vi "SLSC Write Properties.vi"(0 "session in":refnum<k21>, 1 "Stop Updating?":bool, 3 "Detect?":bool[](array[boolean]), 5 "SLSC Module Name":refnum<k21>, 9 "Values":dbl[](array[numeric]), 11 "error in":errorcluster, 12 "SLSC Dynamic Outputs":T1[](array[typedef]), 13 "Change Commands":T1[](array[typedef]), 14 "Command Values":dbl[](array[numeric])) -> (4 "session out":refnum<k21>, 6 "SLSC Module Name":refnum<k21>, 8 "LoopRate(ms)":u32=50, 15 "error out":errorcluster)   [LabVIEW 2020, in "SLSC CD Engine.lvlib"]
uses:
  SLSC CD Engine.lvlib
  SLSC Dynamic Channel.ctl
  SLSC Datatype.ctl
  <vilib>/SLSC/Execute Command.vi
  <vilib>/SLSC/Execute Device Command.vi
  <vilib>/SLSC/Execute Phys Chan Command.vi
  <vilib>/SLSC/Commit Properties for Devices.vi
  <vilib>/SLSC/Set Generic Property (U64).vi
  <vilib>/SLSC/Set Generic Property (I64).vi
  <vilib>/SLSC/Set Generic Property (Bool).vi
  <vilib>/SLSC/Set Generic Property (String).vi
  <vilib>/SLSC/Set Generic Property (U32).vi
  <vilib>/SLSC/Set Generic Property (I32).vi
  <vilib>/SLSC/Set Generic Property (DBL).vi
  <vilib>/SLSC/SLSC.lvlib
  SLSC CD Shared/SLSC CD Shared.lvlib
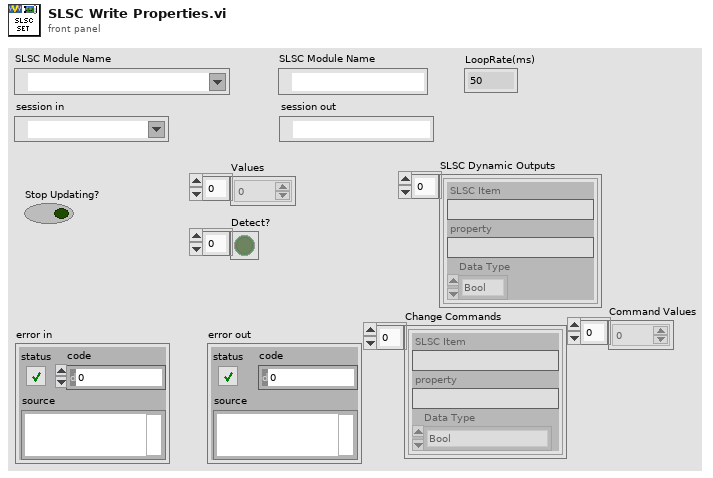
[diagram p1: front panel]
types:
  T1 = typedef "SLSC CD Shared.lvlib/SLSC Dynamic Channel.ctl" = cluster{"SLSC Item":string, "property":string, "Data Type":T2}
  T2 = typedef "SLSC CD Shared.lvlib/SLSC Datatype.ctl" = enum16{"Bool", "Double", "I32", "I64", "String", "U32", "U64"}
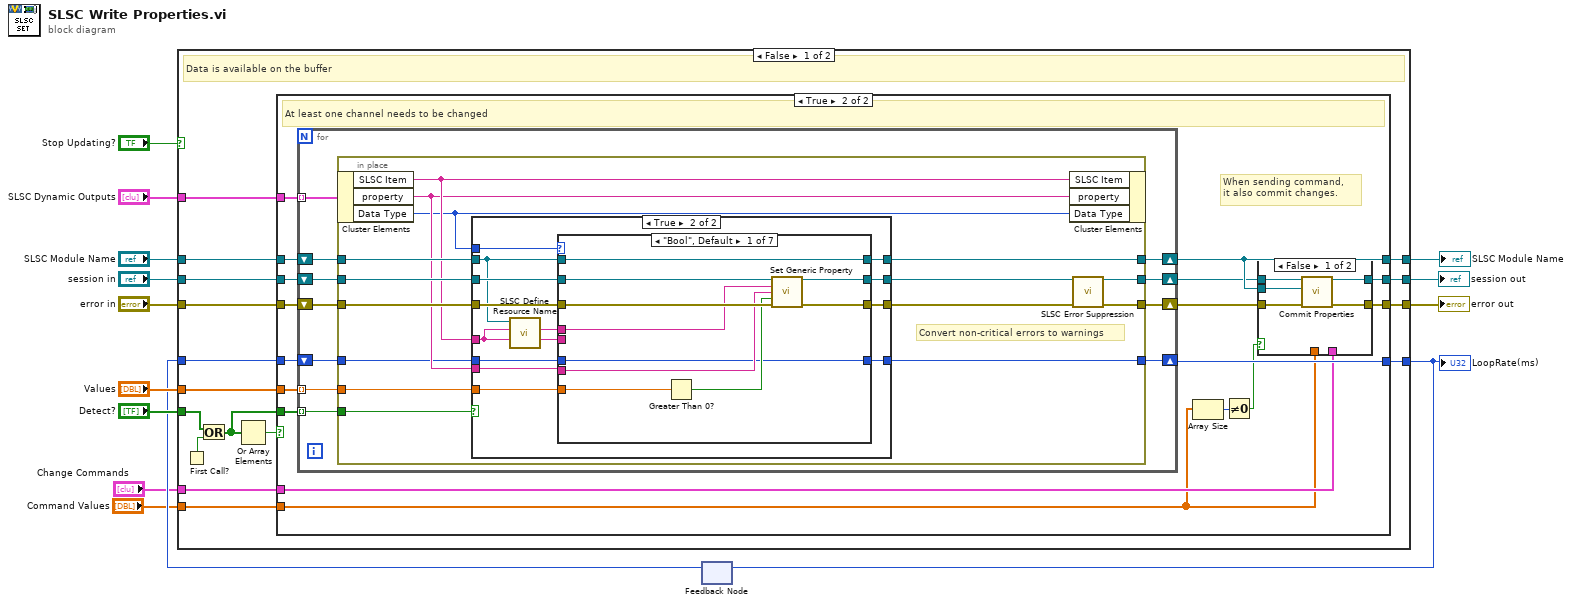
[diagram p0: block diagram]
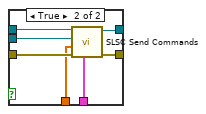
[diagram p3: hidden frame]
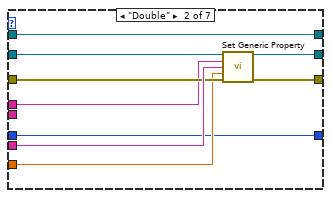
[diagram p5: hidden frame]
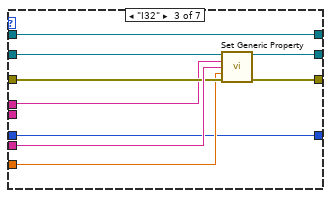
[diagram p6: hidden frame]
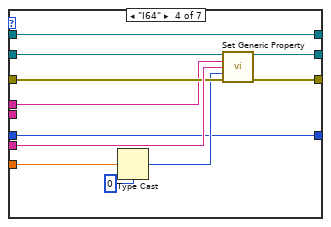
[diagram p7: hidden frame]
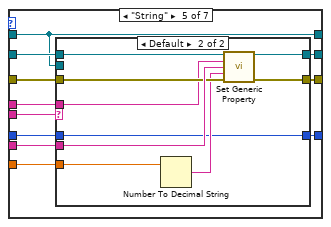
[diagram p8: hidden frame]
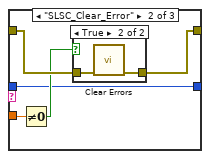
[diagram p10: hidden frame]
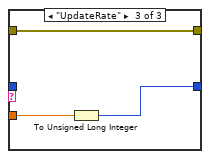
[diagram p12: hidden frame]
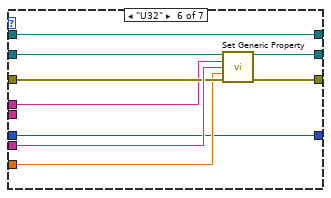
[diagram p13: hidden frame]
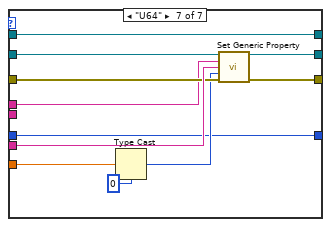
[diagram p14: hidden frame]
diagram:
  n1 = feedback #1() -> (w3:u32)  [unwired: 1 in]
  n2 = case shown="False" "Stop Updating?" {
    tunnel: "error in" -> [w30 w206]
    tunnel: "SLSC Dynamic Outputs" -> [w29 _]
    tunnel: "Values" -> [w28 _]
    tunnel: "session in" -> [w27 w207]
    tunnel: "SLSC Module Name" -> [w26 w208]
    tunnel: [w20 w208] -> w10
    tunnel: [w25 w206] -> w9
    tunnel: [w24 w207] -> w8
    tunnel: "Detect?" -> [w23 _]
    tunnel: [w21 w205] -> w4
    tunnel: w3 -> [w22 w205]
    tunnel: "Change Commands" -> [w18 _]
    tunnel: "Command Values" -> [w17 _]
    frame False {
      # "Data is available on the buffer"
      n3 = First Call?() -> (First Call?: T/F=w15:bool)
      n4 = Or(x=w23, y=w15) -> (x .or. y?=w16:bool[])
      n5 = Or Array Elements(Boolean array=w16) -> (logical OR=w19:bool)
      n6 = case shown="True" w19 {
        tunnel: w30 -> [w32 w51]
        tunnel: w29 -> [_ w50]
        tunnel: w28 -> [_ w49]
        tunnel: w27 -> [w33 w48]
        tunnel: w26 -> [w34 w47]
        tunnel: [w32 w42] -> w25
        tunnel: [w33 w43] -> w24
        tunnel: w16 -> [_ w46]
        tunnel: w22 -> [w31 w45]
        tunnel: [w31 w44] -> w21
        tunnel: [w34 w41] -> w20
        tunnel: w18 -> [_ w40]
        tunnel: w17 -> [_ w35]
        frame False {
          # "Do change detected, bypass write action"
        }
        frame True {
          # "When sending command,\nit also commit changes."
          # "At least one channel needs to be changed"
          n7 = for {
            tunnel: w49 -> [w74] mode=indexing
            tunnel: w50 -> [w67] mode=indexing
            shift-right: [w72] -> w36
            shift-left: w48 -> [w73]
            shift-right: [w71] -> w41
            shift-left: w47 -> [w68]
            tunnel: w46 -> [w66] mode=indexing
            shift-right: [w64] -> w44
            shift-left: w45 -> [w65]
            shift-right: [w69] -> w37
            shift-left: w51 -> [w70]
            n8 = in-place {
              in-place-border: w74 -> [w80]
              in-place-border: w73 -> [w88]
              in-place-border: [w87] -> w72
              in-place-border: [w86] -> w71
              in-place-border: w70 -> [w85]
              in-place-border: [w75] -> w69
              in-place-border: w68 -> [w84]
              in-place-border: w66 -> [w79]
              in-place-border: [w77] -> w64
              in-place-border: w65 -> [w76]
              # "Convert non-critical errors to warnings"
              n9 = in-place-cluster #2(w67) -> ("SLSC Item"=w83:string, "property"=w82:string, "Data Type"=w81:T2)
              n10 = case shown="True" w79 {
                tunnel: w88 -> [w91 w105]
                tunnel: [w91 w104] -> w87
                tunnel: [w92 w103] -> w86
                tunnel: w85 -> [w90 w102]
                tunnel: [w90 w101] -> w78
                tunnel: w84 -> [w92 w100]
                tunnel: w83 -> [_ w98]
                tunnel: w82 -> [_ w97]
                tunnel: w81 -> [_ w96]
                tunnel: w80 -> [_ w95]
                tunnel: [w89 w94] -> w77
                tunnel: w76 -> [w89 w93]
                frame False {
                }
                frame True {
                  n11 = call "SLSC Define Resource Name.vi"("SLSC Item"=w98, "SLSC Module Name"=w100) -> ("Resource"=w99:string)  [unwired: 9 in]
                  n12 = case shown="\"Bool\", Default" w96 {
                    tunnel: w95 -> [w110 w118 w127 w138 w150 w187 w197]
                    tunnel: w105 -> [w115 w124 w133 w144 w155 w193 w204]
                    tunnel: [w114 w123 w132 w143 w154 w192 w203] -> w104
                    tunnel: w97 -> [w107 w122 w131 w142 w153 w191 w202]
                    tunnel: w100 -> [w113 w121 w130 w141 w149 w190 w201]
                    tunnel: [w113 w121 w130 w141 w149 w190 w201] -> w103
                    tunnel: w102 -> [w112 w120 w129 w140 w152 w189 w200]
                    tunnel: [w111 w119 w128 w139 w151 w188 w199] -> w101
                    tunnel: w99 -> [w109 w117 w126 w135 w147 w186 w195]
                    tunnel: w98 -> [_ _ _ _ w148 _ _]
                    tunnel: [w106 w116 w125 w134 w146 w185 w194] -> w94
                    tunnel: w93 -> [w106 w116 w125 w134 w145 w185 w194]
                    frame "Bool", Default {
                      n13 = Greater Than 0?(x=w110) -> (x > 0?=w108:bool)
                      n14 = call-poly <vilib>:"Set Generic Property.vi"("session in"=w115, "resources"=w109, "property"=w107, "property value"=w108, "error in (no error)"=w112) -> ("session out"=w114:refnum<k21>, "error out"=w111:errorcluster)  [unwired: 9 in]
                    }
                    frame "Double" {
                      n15 = call-poly <vilib>:"Set Generic Property.vi"("session in"=w124, "resources"=w117, "property"=w122, "property value"=w118, "error in (no error)"=w120) -> ("session out"=w123:refnum<k21>, "error out"=w119:errorcluster)  [unwired: 9 in]
                    }
                    frame "I32" {
                      n16 = call-poly <vilib>:"Set Generic Property.vi"("session in"=w133, "resources"=w126, "property"=w131, "property value"=w127, "error in (no error)"=w129) -> ("session out"=w132:refnum<k21>, "error out"=w128:errorcluster)  [unwired: 9 in]
                    }
                    frame "I64" {
                      n17 = Type Cast(type=i64 0 ("property value"), x=w138) -> (*(type *) &x=w136:i64)
                      n18 = call-poly <vilib>:"Set Generic Property.vi"("session in"=w144, "resources"=w135, "property"=w142, "property value"=w136, "error in (no error)"=w140) -> ("session out"=w143:refnum<k21>, "error out"=w139:errorcluster)  [unwired: 9 in]
                    }
                    frame "String" {
                      n19 = case shown="Default" w148 {
                        tunnel: w155 -> [w162 w184]
                        tunnel: [w162 w183] -> w154
                        tunnel: w153 -> [w160 w182]
                        tunnel: w149 -> [_ _]
                        tunnel: w152 -> [w158 w181]
                        tunnel: [w159 w180] -> w151
                        tunnel: w150 -> [w161 w179]
                        tunnel: w147 -> [_ w177]
                        tunnel: [w157 w176] -> w146
                        tunnel: w145 -> [w156 w176]
                        frame "Status" {
                          n20 = case shown="Default" w160 {
                            tunnel: w161 -> [_ w167 w174]
                            tunnel: [w164 w168 w175] -> w159
                            tunnel: w158 -> [w164 w169 w175]
                            tunnel: [w163 w165 w173] -> w157
                            tunnel: w156 -> [w163 w165 _]
                            frame Default {
                            }
                            frame "SLSC_Clear_Error" {
                              n21 = Not Equal To 0?(x=w167) -> (x != 0?=w166:bool)
                              n22 = case shown="True" w166 {
                                tunnel: w169 -> [w170 w172]
                                tunnel: [w170 w171] -> w168
                                frame False {
                                }
                                frame True {
                                n23 = call <vilib>:"Clear Errors.vi"("error in (no error)"=w172) -> ("error out"=w171:errorcluster)  [unwired: 5 in, 1 out]
                                }
                              }
                            }
                            frame "UpdateRate" {
                              n24 = To Unsigned Long Integer(number=w174) -> (unsigned 32bit integer=w173:u32)
                            }
                          }
                        }
                        frame Default {
                          n25 = Number To Decimal String(number=w179) -> (decimal integer string=w178:string)  [unwired: 1 in]
                          n26 = call-poly <vilib>:"Set Generic Property.vi"("session in"=w184, "resources"=w177, "property"=w182, "property value"=w178, "error in (no error)"=w181) -> ("session out"=w183:refnum<k21>, "error out"=w180:errorcluster)  [unwired: 9 in]
                        }
                      }
                    }
                    frame "U32" {
                      n27 = call-poly <vilib>:"Set Generic Property.vi"("session in"=w193, "resources"=w186, "property"=w191, "property value"=w187, "error in (no error)"=w189) -> ("session out"=w192:refnum<k21>, "error out"=w188:errorcluster)  [unwired: 9 in]
                    }
                    frame "U64" {
                      n28 = Type Cast(type=u64 0 ("property value"), x=w197) -> (*(type *) &x=w196:u64)
                      n29 = call-poly <vilib>:"Set Generic Property.vi"("session in"=w204, "resources"=w195, "property"=w202, "property value"=w196, "error in (no error)"=w200) -> ("session out"=w203:refnum<k21>, "error out"=w199:errorcluster)  [unwired: 9 in]
                    }
                  }
                }
              }
              n30 = in-place-cluster #2("SLSC Item"=w83, "property"=w82, "Data Type"=w81) -> ()  [unwired: 1 out]
              n31 = call "SLSC Error Suppression.vi"("error in (no error)"=w78) -> ("error out"=w75:errorcluster)  [unwired: 8 in, 1 out]
            }
          }
          n32 = Array Size(array=w35) -> (size(s)=w39:i32)
          n33 = Not Equal To 0?(x=w39) -> (x != 0?=w38:bool)
          n34 = case shown="False" w38 {
            tunnel: w36 -> [w52 w63]
            tunnel: [w54 w62] -> w43
            tunnel: w37 -> [w56 w61]
            tunnel: [w55 w60] -> w42
            tunnel: w41 -> [w53 w59]
            tunnel: w40 -> [_ w58]
            tunnel: w35 -> [_ w57]
            frame False {
              n35 = call-poly <vilib>:"Commit Properties.vi"("session in"=w52, "devices"=w53, "error in (no error)"=w56) -> ("session out"=w54:refnum<k21>, "error out"=w55:errorcluster)  [unwired: 11 in]
            }
            frame True {
              n36 = call "SLSC Send Commands.vi"("SLSC Dynamic Commands"=w58, "error in"=w61, "Values"=w57, "SLSC Module Name"=w59, "session in"=w63) -> ("error out"=w60:errorcluster, "session out"=w62:refnum<k21>)  [unwired: 4 in, 1 out]
            }
          }
        }
      }
    }
    frame True {
      # "No data on the buffer"
    }
  }
  "error out" <- w9
  "session out" <- w8
  "SLSC Module Name" <- w10
  "LoopRate(ms)" <- w4
  n37 = feedback-in #1(w4) -> ()
